vi "Semantic_DialoguePyPl_Array_Msg.vi"(8 "error in (no error)":errorcluster caption="错误输入（无错误）", 10 "值(信号)":T2, 11 "States.lvlib:Voice.lvclass":refnum<class "Voice.lvclass">) -> (0 "error out":errorcluster caption="错误输出", 3 "Process State out":refnum<class "State Actor.lvclass">)   [LabVIEW 2014, in "States.lvlib" / "Voice.lvclass"]
uses:
  Voice.lvclass
  ctl/Semantic_Voice_Array.ctl
  <vilib>/NI/Actors/State Actor/State Actor/State Actor.lvclass
  <vilib>/ActorFramework/Message Enqueuer/Message Enqueuer.lvclass/Message Enqueuer.ctl
  <vilib>/ActorFramework/Message Enqueuer/Enqueue.vi
  Global_var/Global_var.vi
  <vilib>/ActorFramework/Message Priority Queue/Priority Enqueue.vi
  Dialogue_lib/DialogueActor/Dialogue.lvclass
panel:
  out "机器人语音指令数据簇数组(Voice)":T1(array[cluster])
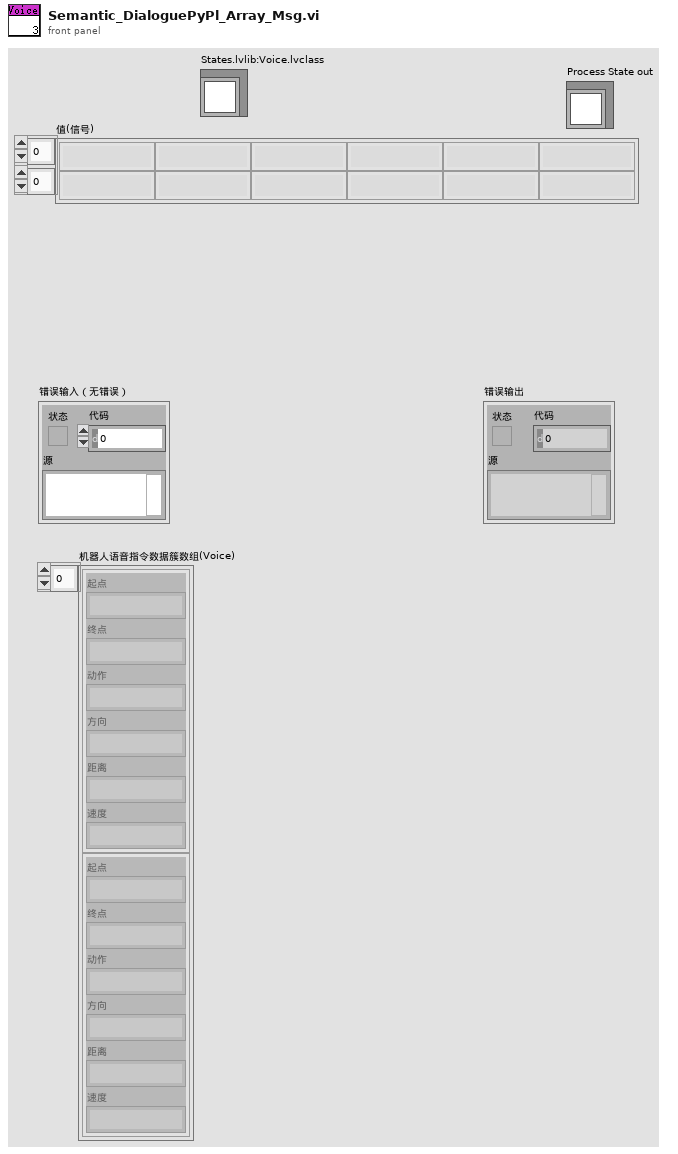
[diagram p1: front panel]
types:
  T1 = cluster{"起点":string, "终点":string, "动作":string, "方向":string, "距离":string, "速度":string}[]
  T2 = typedef "Semantic_Voice_Array.ctl" = string[][]
  T3 = cluster{"rot_z_max":dbl, "lin_x_max":dbl, "rot_z_min":dbl, "lin_x_min":dbl}
  T4 = cluster{"pose_X":dbl, "pose_Y":dbl, "pose_z":dbl, "pose_rot":dbl, "force_bool":bool}
  T5 = cluster{"pose_X":dbl, "pose_Y":dbl, "pose_z":dbl, "pose_rot":dbl, "force_bool":bool}[]
  T6 = cluster{"now_pose_X":dbl, "now_pose_Y":dbl, "now_pose_Rot_deg":dbl}
  T7 = cluster{"起点":string, "终点":string, "动作":string, "方向":string, "距离":string, "速度":string}
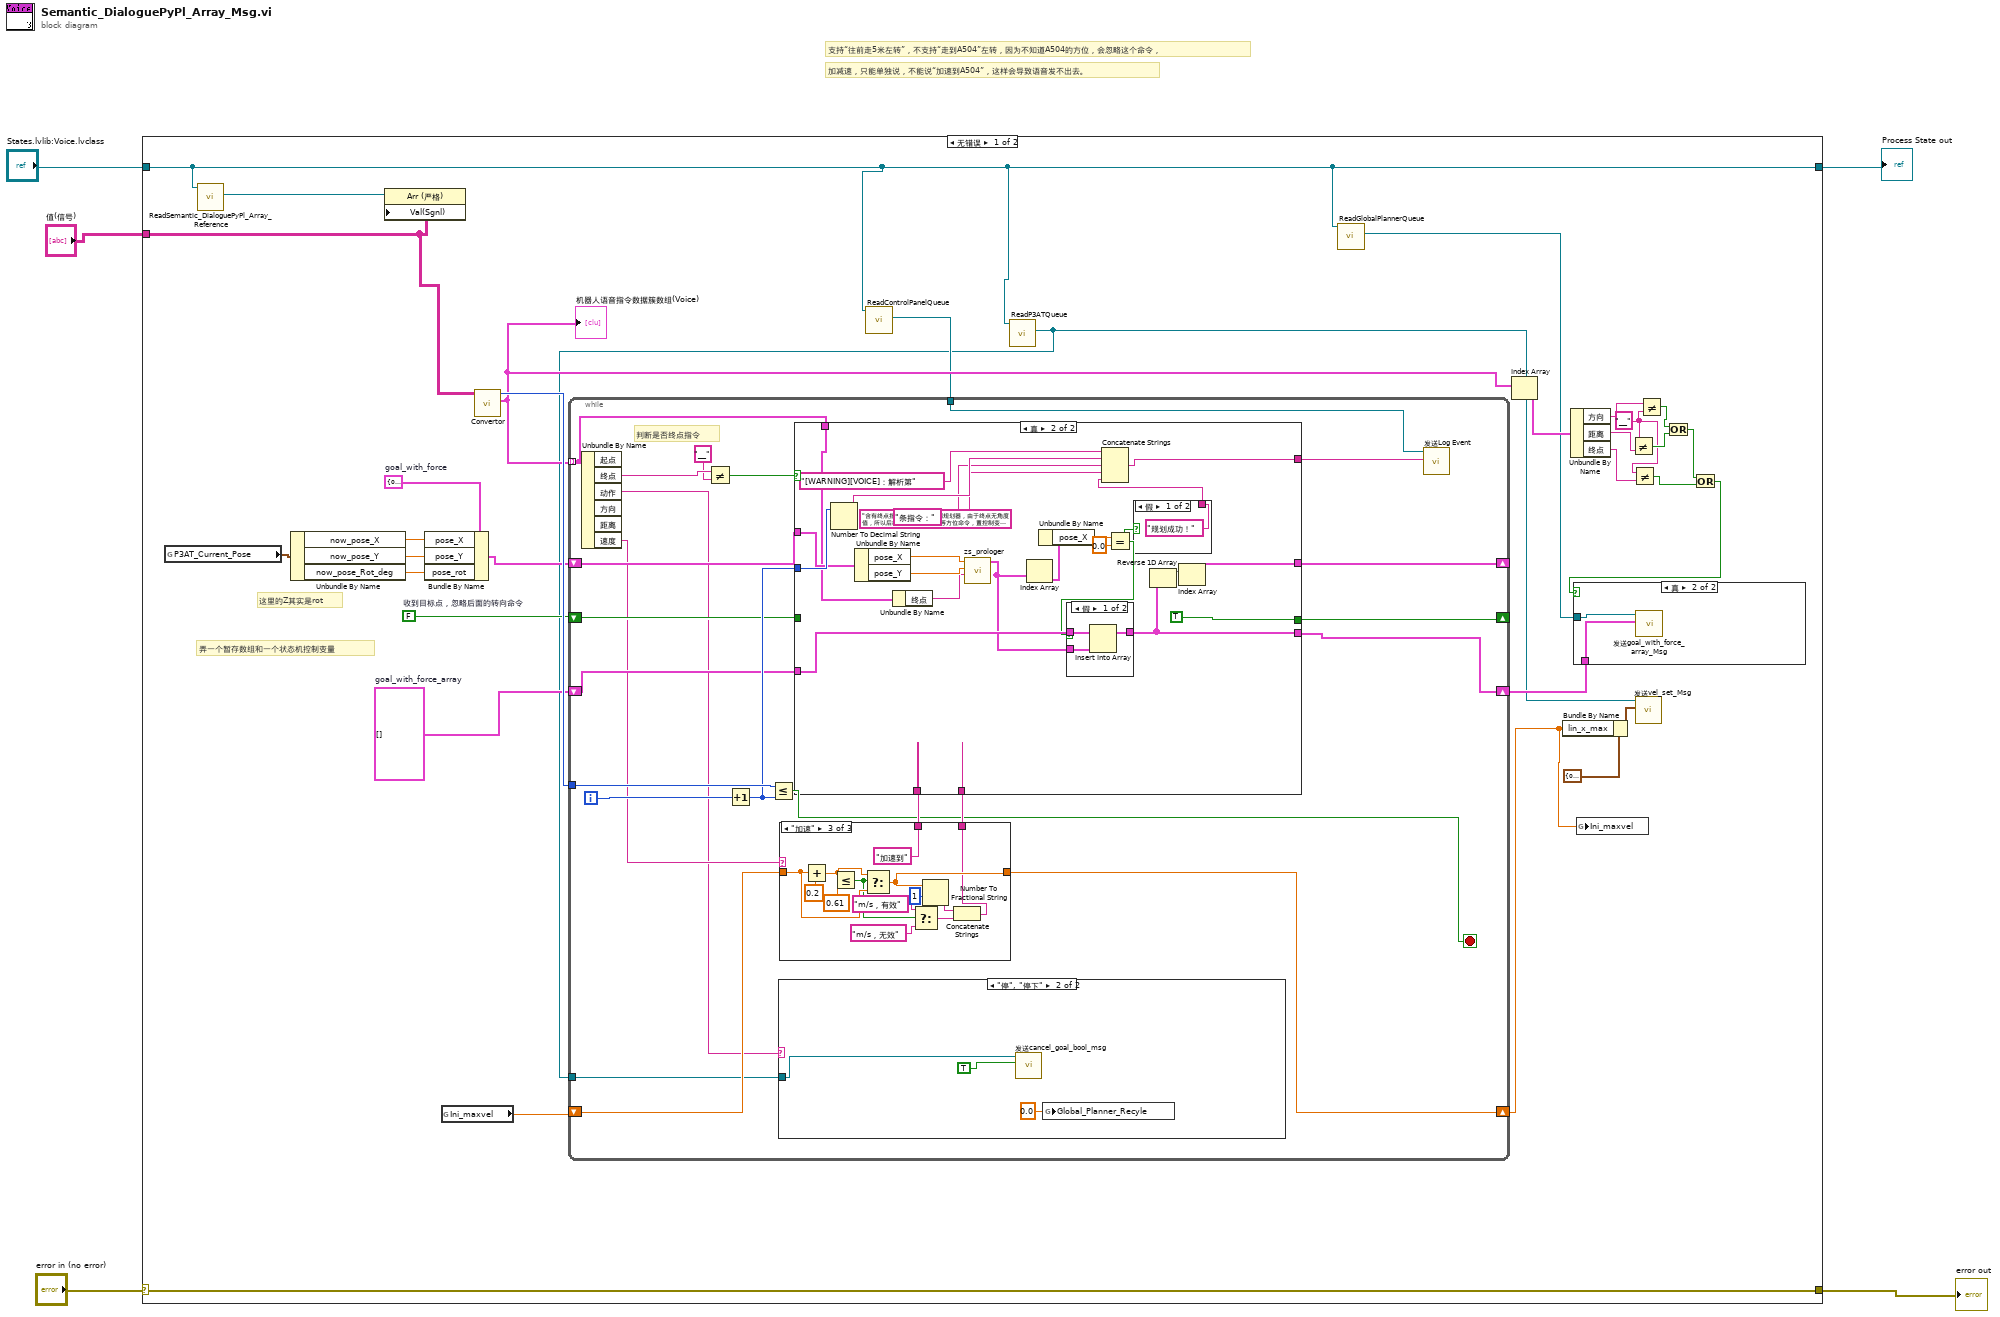
[diagram p0: block diagram]
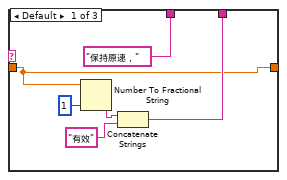
[diagram p4: hidden frame]
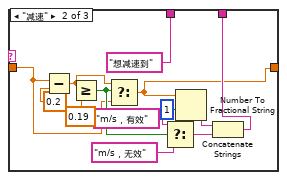
[diagram p5: hidden frame]
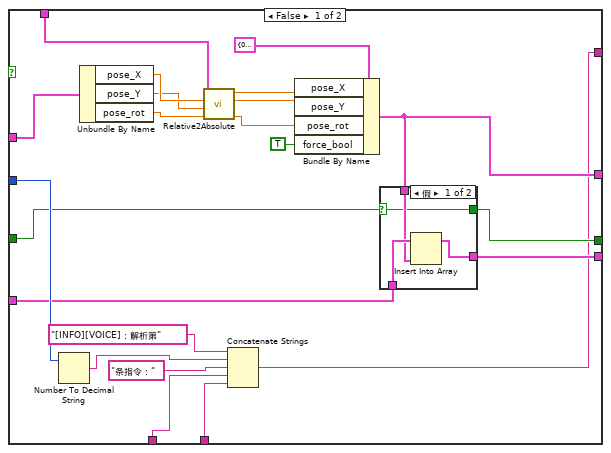
[diagram p6: hidden frame]
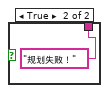
[diagram p9: hidden frame]
diagram:
  # "加减速，只能单独说，不能说“加速到A504”，这样会导致语音发不出去。"
  # "支持“往前走5米左转”，不支持“走到A504”左转，因为不知道A504的方位，会忽略这个命令，"
  n1 = case shown="无错误" "error in (no error)" {
    selector: "error in (no error)" -> [w37 w154]
    tunnel: [w37 w154] -> w4
    tunnel: [w15 w155] -> w2
    tunnel: "States.lvlib:Voice.lvclass" -> [w15 w155]
    tunnel: "值(信号)" -> [w27 _]
    frame No Error {
      w10 = "__"
      w28 = T4 {"pose_X"=0.0, "pose_Y"=0.0, "pose_z"=0.0, "pose_rot"=0.0, "force_bool"=FALSE}  # goal_with_force
      w29 = T5 []  # goal_with_force_array
      w30 = FALSE  # 收到目标点，忽略后面的转向命令
      # "这里的Z其实是rot"
      # "弄一个暂存数组和一个状态机控制变量"
      n2 = global read "Global_var.vi" "P3AT_Current_Pose"() -> (w26:T6)
      n3 = call-dynamic "ReadSemantic_DialoguePyPl_Array_Reference.vi"("CoordinatorState输入"=w15) -> ("Semantic_DialoguePyPl_Array_Reference"=w36:refnum<vi>)  [unwired: 8 in, 2 out]
      n4 = Unbundle By Name(w26) -> ("now_pose_X"=w34:dbl, "now_pose_Y"=w33:dbl, "now_pose_Rot_deg"=w32:dbl)
      n5 = property class="Arr (严格)"(reference=w36, "Val(Sgnl)"=w27) -> ()  [unwired: 1 in, 2 out]
      n6 = Bundle By Name(cluster=w28, "pose_X"=w34, "pose_Y"=w33, "pose_rot"=w32) -> (w31:T4)
      n7 = global read "Global_var.vi" "Ini_maxvel"() -> (w25:dbl)
      n8 = call "Convertor.vi"("格式化机器人指令"=w27) -> ("机器人语音指令数据簇数组(Voice)"=w18:T1, "命令个数"=w35:i32)  [unwired: 8 in, 1 out]
      "机器人语音指令数据簇数组(Voice)" <- w18
      n9 = call-dynamic "ReadControlPanelQueue.vi"("CoordinatorState输入"=w15) -> ("操作者框架:消息待入队列"=w16:refnum<class "Message Enqueuer.lvclass">)  [unwired: 8 in, 2 out]
      n10 = call-dynamic "ReadP3ATQueue.vi"("CoordinatorState输入"=w15) -> ("操作者框架:消息待入队列"=w6:refnum<class "Message Enqueuer.lvclass">)  [unwired: 8 in, 2 out]
      n11 = while {
        tunnel: w18 -> [w61] mode=indexing
        shift-right: [w50] -> _
        shift-left: w31 -> [w52]
        tunnel: w35 -> [w59]
        shift-right: [w55] -> w17
        shift-left: w25 -> [w57]
        shift-right: [w47] -> w13
        shift-left: w29 -> [w51]
        shift-right: [w48] -> _
        shift-left: w30 -> [w49]
        tunnel: w16 -> [w42]
        tunnel: w6 -> [w40]
        i -> [w60]
        stop <- w53 stop-if-true
        # "判断是否终点指令"
        n12 = Unbundle By Name(w61) -> ("终点"=w62:string, "动作"=w41:string, "速度"=w46:string)  [unwired: 3 out]
        n13 = Not Equal?(x=w62, y="__") -> (x != y?=w44:bool)
        n14 = Increment(x=w60) -> (x+1=w58:i32)
        n15 = Less Or Equal?(x=w59, y=w58) -> (x <= y?=w53:bool)
        n16 = case shown="\"停\", \"停下\"" w41 {
          tunnel: w40 -> [_ w64]
          frame "假", Default {
          }
          frame "停", "停下" {
            n17 = call "发送cancel_goal_bool_msg.vi"("值(信号)"=TRUE, "消息待入队列"=w64) -> ()  [unwired: 8 in, 2 out]
            n18 = global write "Global_var.vi" "Global_Planner_Recyle"(0.0 ("Global_Planner_Recyle")) -> ()
          }
        }
        n19 = case shown="\"加速\"" w46 {
          tunnel: w57 -> [w67 w73 w93]
          tunnel: ["保持原速，" ("Event Text") "想减速到" ("Event Text") "加速到" ("Event Text")] -> w56
          tunnel: [w67 w74 w88] -> w55
          tunnel: [w68 w75 w87] -> w54
          frame Default {
            n20 = Number To Fractional String(number=w67, precision (6)=i16 1 ("精度(6)")) -> (F-format string=w70:string)  [unwired: 2 in]
            n21 = Concatenate Strings(w70, "有效" ("Event Text")) -> (w68:string)
          }
          frame "减速" {
            n22 = Subtract(x=w73, y=0.2) -> (x-y=w82:dbl)
            n23 = Greater Or Equal?(x=w82, y=0.19) -> (x >= y?=w81:bool)
            n24 = Select(t=w82, s=w81, f=w73) -> (s? t:f=w74:dbl)
            n25 = Select(t="m/s，有效" ("Event Text"), s=w81, f="m/s，无效" ("Event Text")) -> (s? t:f=w78:string)
            n26 = Number To Fractional String(number=w74, precision (6)=i16 1 ("精度(6)")) -> (F-format string=w77:string)  [unwired: 2 in]
            n27 = Concatenate Strings(w77, w78) -> (w75:string)
          }
          frame "加速" {
            n28 = Add(x=w93, y=0.2) -> (x+y=w94:dbl)
            n29 = Less Or Equal?(x=w94, y=0.61) -> (x <= y?=w86:bool)
            n30 = Select(t=w94, s=w86, f=w93) -> (s? t:f=w88:dbl)
            n31 = Select(t="m/s，有效" ("Event Text"), s=w86, f="m/s，无效" ("Event Text")) -> (s? t:f=w90:string)
            n32 = Number To Fractional String(number=w88, precision (6)=i16 1 ("精度(6)")) -> (F-format string=w89:string)  [unwired: 2 in]
            n33 = Concatenate Strings(w89, w90) -> (w87:string)
          }
        }
        n34 = case shown="真" w44 {
          tunnel: w61 -> [w119 w139]
          tunnel: [w104 w133] -> w50
          tunnel: w52 -> [w112 w142]
          tunnel: w58 -> [w115 w147]
          tunnel: w56 -> [w114 _]
          tunnel: w54 -> [w113 _]
          tunnel: w51 -> [w105 w137]
          tunnel: [w100 w135] -> w47
          tunnel: w49 -> [w102 _]
          tunnel: [w101 TRUE] -> w48
          tunnel: [w98 w126] -> w43
          frame False {
            n35 = Number To Decimal String(number=w115) -> (decimal integer string=w117:string)  [unwired: 1 in]
            n36 = Unbundle By Name(w112) -> ("pose_X"=w111:dbl, "pose_Y"=w110:dbl, "pose_rot"=w109:dbl)
            n37 = call "Relative2Absolute.vi"("机器人语音指令数据簇"=w119, "now_pose_X"=w111, "now_pose_Y"=w110, "now_pose_Rot_deg"=w109) -> ("x"=w108:dbl, "y"=w107:dbl, "Rot_deg"=w106:dbl)  [unwired: 4 in]
            n38 = Concatenate Strings("[INFO][VOICE]：解析第" ("Event Text"), w117, "条指令：" ("Event Text"), w114, w113) -> (w98:string)
            n39 = Bundle By Name(cluster=T4 {"pose_X"=0.0, "pose_Y"=0.0, "pose_z"=0.0, "pose_rot"=0.0, "force_bool"=FALSE} ("goal_with_force"), "pose_X"=w108, "pose_Y"=w107, "pose_rot"=w106, "force_bool"=TRUE) -> (w104:T4)
            n40 = case shown="假" w102 {
              selector: w102 -> [w121 w125]
              tunnel: w105 -> [w123 w124]
              tunnel: w104 -> [w122 _]
              tunnel: [w121 w125] -> w101
              tunnel: [w120 w124] -> w100
              frame False {
                n41 = Insert Into Array(array=w123, new element=w122) -> (w120:T5)  [unwired: 1 in]
              }
              frame True {
              }
            }
          }
          frame True {
            n42 = Number To Decimal String(number=w147) -> (decimal integer string=w145:string)  [unwired: 1 in]
            n43 = Unbundle By Name(w142) -> ("pose_X"=w141:dbl, "pose_Y"=w140:dbl)
            n44 = Unbundle By Name(w139) -> ("终点"=w138:string)
            n45 = call "zs_prologer.vi"("goal_node"=w138, "y"=w140, "x"=w141) -> ("goal_array"=w132:T5)  [unwired: 6 in]
            n46 = Index Array(array=w132) -> (element=w131:T4)  [unwired: 1 in]
            n47 = Unbundle By Name(w131) -> ("pose_X"=w130:dbl)
            n48 = Equal?(x=w130, y=0.0) -> (x = y?=w127:bool)
            n49 = case shown="假" w127 {
              tunnel: w137 -> [w150 w151]
              tunnel: [w149 w151] -> w135
              tunnel: w132 -> [w148 _]
              frame False {
                n50 = Insert Into Array(array=w150, new element=w148) -> (w149:T5)  [unwired: 1 in]
              }
              frame True {
              }
            }
            n51 = case shown="假" w127 {
              tunnel: ["规划成功！" "规划失败！"] -> w128
              frame False {
              }
              frame True {
              }
            }
            n52 = Concatenate Strings("[WARNING][VOICE]：解析第" ("Event Text"), w145, "条指令：" ("Event Text"), "含有终点指令元素，调用全局规划器，由于终点无角度值，所以后续无法执行“左转”等方位命令，置控制变量，忽略此“转向命令”\n" ("Event Text"), w128) -> (w126:string)
            n53 = Reverse 1D Array(array=w135) -> (reversed array=w134:T5)
            n54 = Index Array(array=w134) -> (element=w133:T4)  [unwired: 1 in]
          }
        }
        n55 = call "发送Log Event.vi"("Event Text"=w43, "消息待入队列"=w42) -> ()  [unwired: 8 in, 2 out]
      }
      n56 = call-dynamic "ReadGlobalPlannerQueue.vi"("CoordinatorState输入"=w15) -> ("操作者框架:消息待入队列"=w14:refnum<class "Message Enqueuer.lvclass">)  [unwired: 8 in, 2 out]
      n57 = Index Array(array=w18) -> (element=w22:T7)  [unwired: 1 in]
      n58 = Bundle By Name(cluster=T3 {"rot_z_max"=0.0, "lin_x_max"=0.0, "rot_z_min"=0.0, "lin_x_min"=0.0} ("vel_set"), "lin_x_max"=w17) -> (w23:T3)
      n59 = Unbundle By Name(w22) -> ("方向"=w21:string, "距离"=w20:string, "终点"=w11:string)
      n60 = global write "Global_var.vi" "Ini_maxvel"(w17) -> ()
      n61 = Not Equal?(x=w10, y=w20) -> (x != y?=w12:bool)
      n62 = Not Equal?(x=w10, y=w11) -> (x != y?=w8:bool)
      n63 = call "发送vel_set_Msg.vi"("值(信号)"=w23, "消息待入队列"=w6) -> ()  [unwired: 8 in, 2 out]
      n64 = Not Equal?(x=w21, y=w10) -> (x != y?=w19:bool)
      n65 = Or(x=w19, y=w12) -> (x .or. y?=w7:bool)
      n66 = Or(x=w7, y=w8) -> (x .or. y?=w9:bool)
      n67 = case shown="真" w9 {
        tunnel: w14 -> [_ w38]
        tunnel: w13 -> [_ w39]
        frame False {
        }
        frame True {
          n68 = call "发送goal_with_force_array_Msg.vi"("值(信号)"=w39, "消息待入队列"=w38) -> ()  [unwired: 8 in, 2 out]
        }
      }
    }
    frame Error {
    }
  }
  "error out" <- w4
  "Process State out" <- w2
